vi "VM Spy - MCListBox ColHdl sorting control.vi"(10 "sort column":i32=-2, 11 "Total columns":i32=2) -> (1 "reversed order":bool, 2 "column to sort":i32, 4 "update required":bool)   [LabVIEW 2021]
doc: "::: CalcExpress Toolkit :::\nCopyright (c) 2000-2026 Konstantin Shifershteyn. All rights reserved."
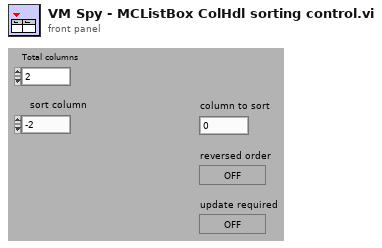
[diagram p1: front panel]
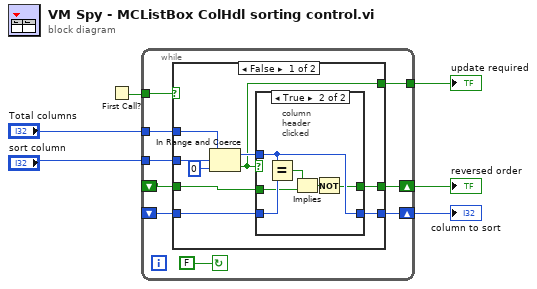
[diagram p0: block diagram]
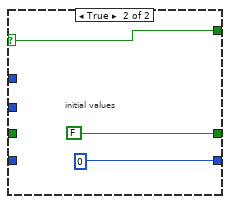
[diagram p3: hidden frame]
diagram:
  n1 = First Call?() -> (First Call?: T/F=w5:bool)
  n2 = while {
    shift-right: [w13] -> w3
    shift-left: _ -> [w10]
    tunnel: w5 -> [w14]
    shift-right: [w12] -> w4
    shift-left: _ -> [w9]
    tunnel: "sort column" -> [w11]
    tunnel: [w8] -> w2
    tunnel: "Total columns" -> [w7]
    stop <- FALSE continue-if-true
    n3 = case shown="False" w14 {
      selector: w14 -> [_ w33]
      tunnel: [w22 0 ("t")] -> w13
      tunnel: [w20 FALSE] -> w12
      tunnel: w11 -> [w23 _]
      tunnel: w10 -> [w21 _]
      tunnel: w9 -> [w19 _]
      tunnel: [w17 w33] -> w8
      tunnel: w7 -> [w16 _]
      frame False {
        n4 = In Range and Coerce(upper limit=w16, x=w23, lower limit=0) -> (coerced(x)=w18:i32, In Range?=w17:bool)
        n5 = case shown="True" w17 {
          tunnel: [w26 w31] -> w22
          tunnel: w21 -> [w26 w32]
          tunnel: [w25 w27] -> w20
          tunnel: w19 -> [w25 w30]
          tunnel: w18 -> [_ w31]
          frame False {
          }
          frame True {
            # "column\nheader\nclicked"
            n6 = Equal?(x=w31, y=w32) -> (x = y?=w29:bool)
            n7 = Implies(1:w30, 2:w29) -> (0:w28:bool)
            n8 = Not(x=w28) -> (.not. x?=w27:bool)
          }
        }
      }
      frame True {
        # "initial values"
      }
    }
  }
  "column to sort" <- w3
  "reversed order" <- w4
  "update required" <- w2
